vi "Handle Error.vi"(8 "error in (no error)":errorcluster, 11 "ZM-ROOT-root in":refnum<class "ZM-ROOT-root.lvclass">) -> (0 "error out":errorcluster, 2 "stop actor?":bool=TRUE, 3 "ZM-ROOT-root out":refnum<class "ZM-ROOT-root.lvclass">)   [LabVIEW 2020, in "ZM-ROOT-root.lvlib" / "ZM-ROOT-root.lvclass"]
doc: "Handle Error override of the root: Call Parent first (it clears error 43 from a normal stop), then ZM-ROOT-evaluateError. Error-handling plan: none yet; evaluateError passes the error on, so an error stops the root and, through AF's Stop Core, the whole tree."
uses:
  ZM-ROOT-root.lvclass
  <vilib>/ActorFramework/Actor/Actor.lvclass
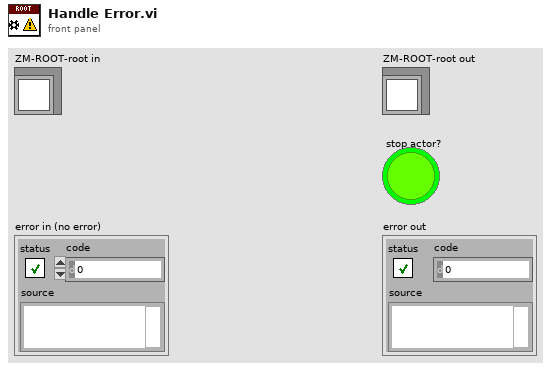
[diagram p1: front panel]
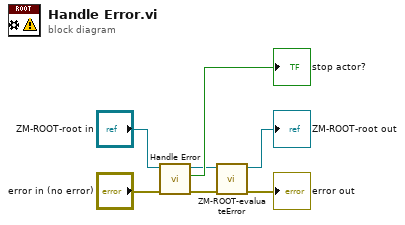
[diagram p0: block diagram]
diagram:
  n1 = call-parent "Handle Error.vi"("error in (no error)"="error in (no error)", "Actor in"="ZM-ROOT-root in") -> ("error out"=w1:errorcluster, "stop actor?"=→"stop actor?":bool, "Actor out"=w3:refnum<class "ZM-ROOT-root.lvclass">)  [unwired: 7 in]
  n2 = call "ZM-ROOT-evaluateError.vi"("error in (no error)"=w1, "ZM-ROOT-root in"=w3) -> ("error out"=→"error out":errorcluster, "ZM-ROOT-root out"=→"ZM-ROOT-root out":refnum<class "ZM-ROOT-root.lvclass">)  [unwired: 7 in, 1 out]
